vi "Close.vi"(8 "error in (no error)":errorcluster, 11 "Tool in":refnum<class "MockTool.lvclass">) -> (0 "error out":errorcluster, 3 "Tool out":refnum<class "MockTool.lvclass">)   [LabVIEW 2017, in "MockTool.lvclass"]
uses:
  MockTool.lvclass
  Server/ITool/ITool.lvclass
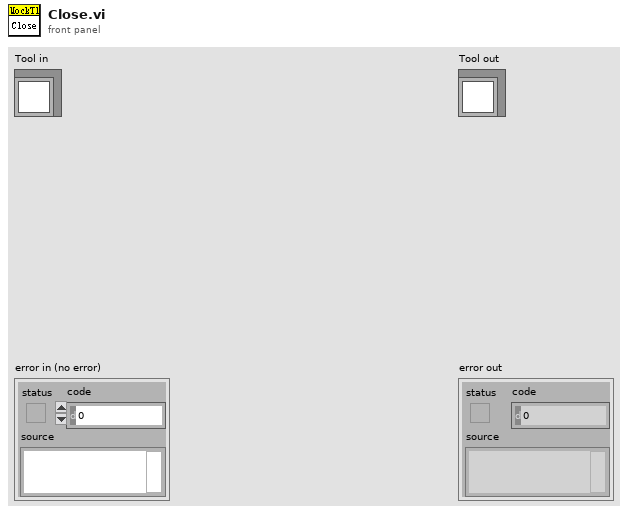
[diagram p1: front panel]
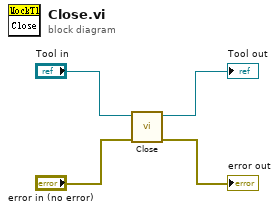
[diagram p0: block diagram]
diagram:
  n1 = call-parent "Close.vi"("error in (no error)"="error in (no error)", "Tool in"="Tool in") -> ("error out"=→"error out":errorcluster, "Tool out"=→"Tool out":refnum<class "MockTool.lvclass">)  [unwired: 8 in]
